vi "Main.vi"(11 "Module Admin":refnum<class "Delacor_lib_QMH_Cloneable Module Admin.lvclass">) -> ()   [LabVIEW 2026, in "Core.lvlib"]
doc: "This template is based off of the Queued Message Handler design pattern and the Queued Message Handler project template that ships with LabVIEW.\n\nThe main difference is that the queue is private to this module and communication between modules is performed via Broadcast and Request events.\n\nRequest events are wrapped in public API methods and are handled in the Event Handling Loop (EHL) of this VI. Any module can register for Broadcast events sent by this module. The EHL generates messages based on user interface actions.\n\nThe Message Handling Loop (MHL) processes messages generated by the EHL, or by other messages. The messages are string values, so new messages can be added easily to the Message Cases case structure in the MHL. Each message cluster can also provide an optional value for Message Data, which is a variant that can be converted to whatever message-specific data is required.\n_____\nBased on DQMH Dev Tools: Project Template 7.1.2.1547."
uses:
  Core.lvlib
  <vilib>/Delacor/Delacor QMH/Libraries/Cloneable Module Admin_class/Delacor_lib_QMH_Cloneable Module Admin.lvclass
  C:/Program Files/National Instruments/LabVIEW 2026/vi.lib/Delacor/Delacor QMH/Libraries/Module Admin_class/Delacor_lib_QMH_Module Admin.lvclass
  Module Data--cluster.ctl
  <vilib>/Delacor/Delacor QMH/Libraries/Message Queue_class/Delacor_lib_QMH_Message Queue.lvclass/Delacor_lib_QMH_Message Queue.ctl
  <vilib>/Delacor/Delacor QMH/Libraries/Cloneable Module Admin_class/Delacor_lib_QMH_Cloneable Module Admin.lvclass/Delacor_lib_QMH_Cloneable Module Admin.ctl
  Stop Argument--cluster.ctl
  <vilib>/Delacor/Delacor QMH/Libraries/Module Admin_class/Delacor_lib_QMH_Module Admin.lvclass/Delacor_lib_QMH_Module Admin.ctl
  LaunchReplayModule Argument--cluster.ctl
  Set Record Run ID Argument--cluster.ctl
  Record Run ID Argument--cluster.ctl
  Record Run ID (Reply Payload)--cluster.ctl
  <vilib>/Utility/miscctls.llb/LVPointTypeDef.ctl
  <vilib>/Delacor/Delacor QMH/Libraries/Message Queue_class/Delacor_lib_QMH_Enqueue Message (Single).vi
  <vilib>/Delacor/Delacor QMH/Libraries/Cloneable Module Admin_class/Delacor_lib_QMH_Get Module ID.vi
  <vilib>/Delacor/Delacor QMH/Libraries/Module Admin_class/Delacor_lib_QMH_Get External Launch.vi
  <vilib>/Delacor/Delacor QMH/Libraries/Message Queue_class/Delacor_lib_QMH_Message Queue.lvclass
  Launcher/Launcher.lvlib
panel:
  out "error out":errorcluster
  out "Status":string
  in  "Simulate EHL Error":bool
  in  "Simulate MHL Error":bool
  # "Other processes communicate with this Module via its Public API (wrappers for its Request Events).\n\nThis Module communicates with other processes via its Broadcast Events.\nAny process that wants to receive these messages can register for this module's Broadcast events."
  # "This template is for the DQMH framework. See the block diagram for more information on how to use this template."
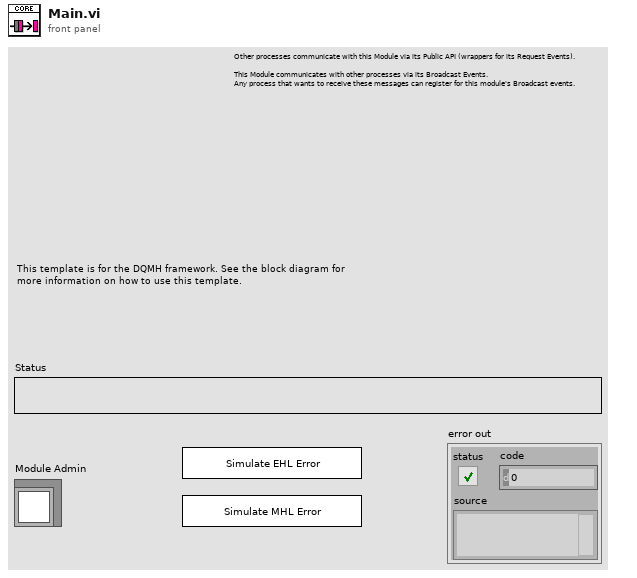
[diagram p1: front panel]
types:
  T1 = typedef "Core.lvlib/Request Events--cluster.ctl" = cluster{"Stop Module":refnum<user-event>, "Show Panel":refnum<user-event>, "Hide Panel":refnum<user-event>, "Show Diagram":refnum<user-event>, "Get Module Execution Status":refnum<user-event>, "Resubscribe to Cloneable":refnum<user-event>, "LaunchReplayModule":refnum<user-event>, "Local Instance":T2, "Record Run ID":refnum<user-event>}
  T2 = typedef "Core.lvlib/Local Instance Request Events--cluster.ctl" = cluster{"Set Record Run ID":refnum<user-event>}
  T3 = typedef "Launcher.lvlib/Broadcast Events--cluster.ctl" = cluster{"Module Did Init":refnum<user-event>, "Status Updated":refnum<user-event>, "Error Reported":refnum<user-event>, "Module Did Stop":refnum<user-event>, "Update Module Execution Status":refnum<user-event>, "Start Capture Detection Loop":refnum<user-event>, "Benchmark Started":refnum<user-event>, "Broadcast number of frames and run ID":refnum<user-event>}
  T4 = typedef "Core.lvlib/Module Data--cluster.ctl" = cluster{"Status":string, "Module ID Recorder":i32, "Record Run ID":string, "Replay Run ID":string}
  T5 = enum32{"invalid lock state", "Not Locked", "Locked (No Password)", "Password-protected"}
  T6 = typedef "Core.lvlib/Stop Argument--cluster.ctl" = cluster{"Module ID":i32, "Origin":string, "Exit via Stop Module Req?":bool, "Wait for Module to stop?":bool}
  T7 = typedef "Core.lvlib/LaunchReplayModule Argument--cluster.ctl" = cluster{"Module ID":i32, "Run ID":string}
  T8 = typedef "Core.lvlib/Set Record Run ID Argument--cluster.ctl" = cluster{"Module ID":i32, "Record Run ID":string}
  T9 = typedef "Core.lvlib/Record Run ID Argument--cluster.ctl" = cluster{"Module ID":i32, "Record Run ID":string, "Wait Notifier":refnum<notifier>, "wait for reply":bool}
  T10 = typedef "LVPointTypeDef.ctl" = cluster{"Horizontal":i16, "Vertical":i16}
  T11 = enum32{"Invalid", "Standard", "Closed", "Hidden", "Minimized", "Maximized"}
  T12 = typedef "Core.lvlib/Record Run ID (Reply Payload)--cluster.ctl" = cluster{"Module ID":i32, "error":errorcluster}
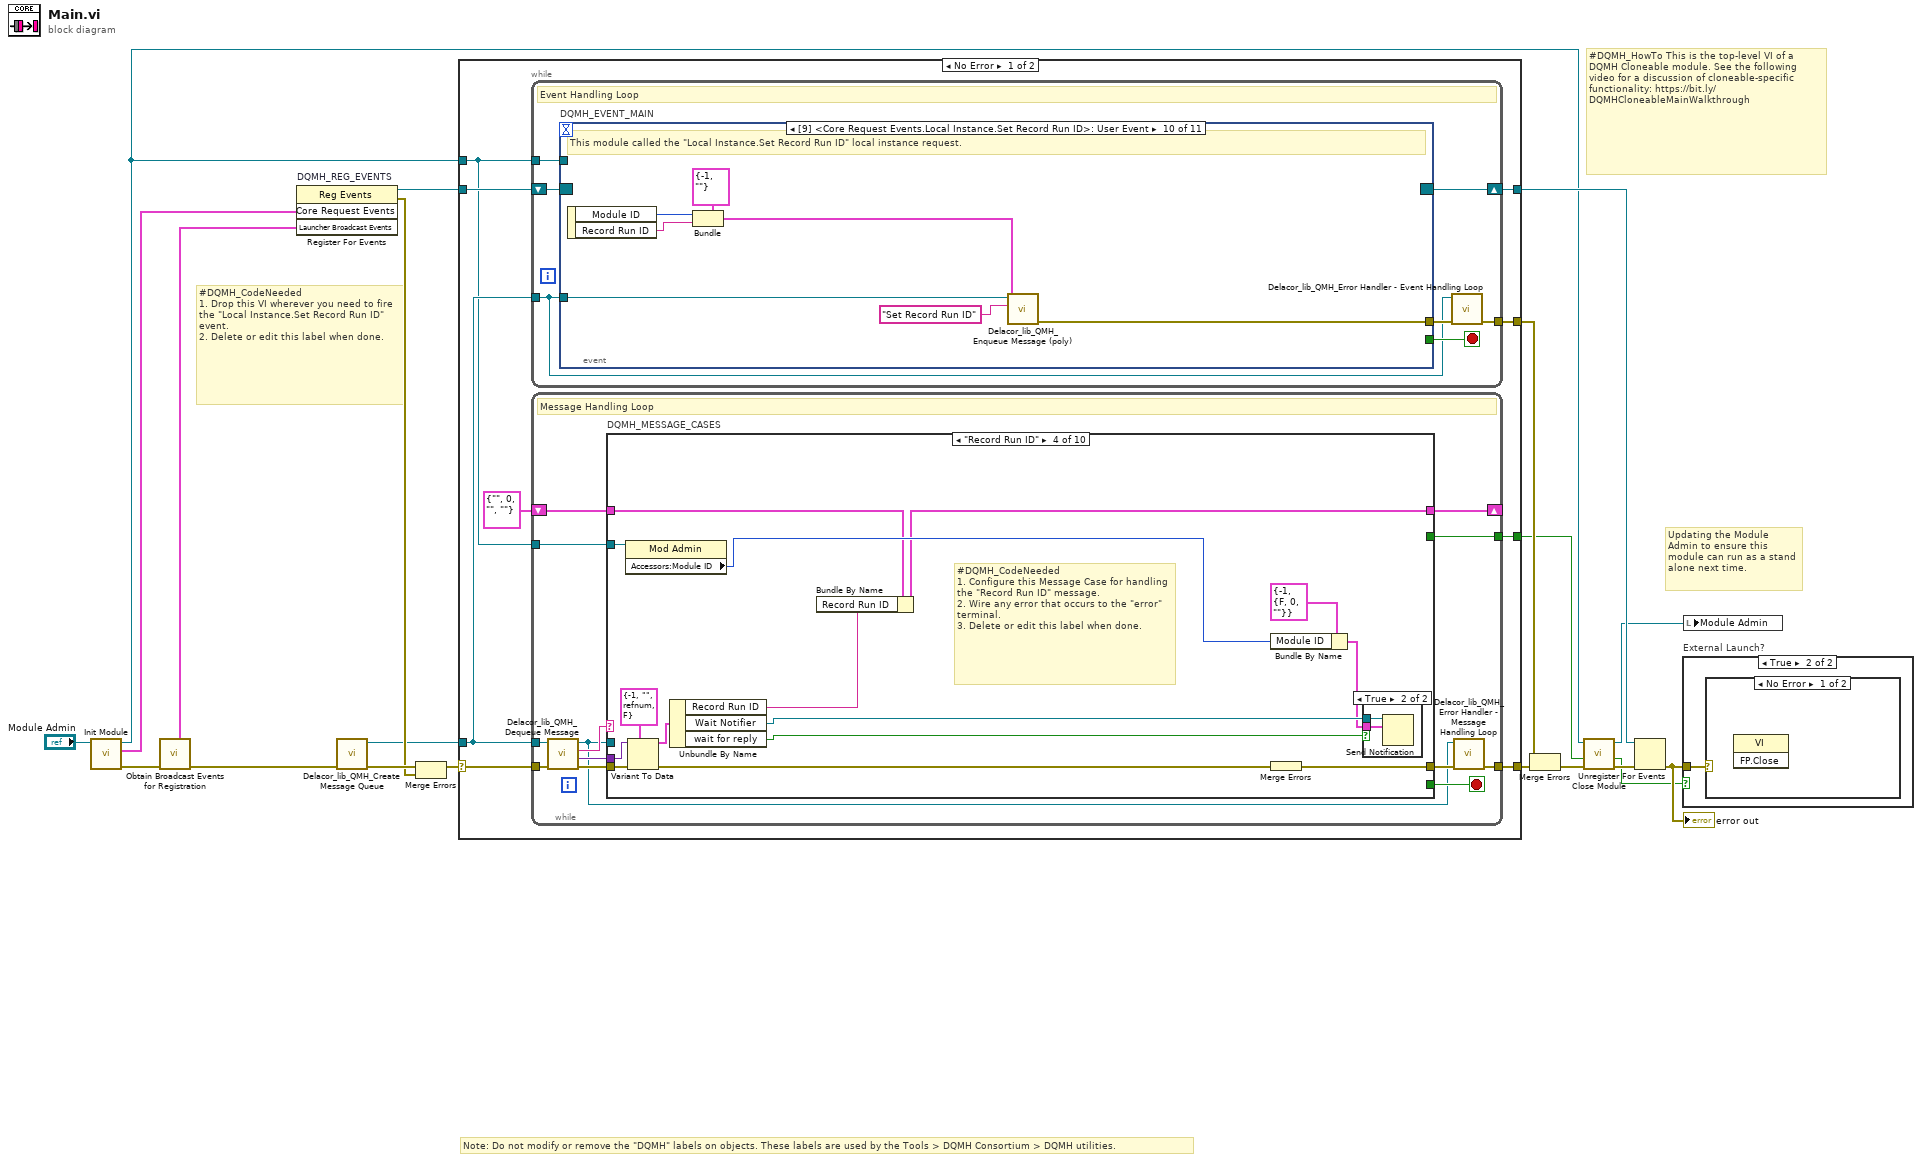
[diagram p0: block diagram]
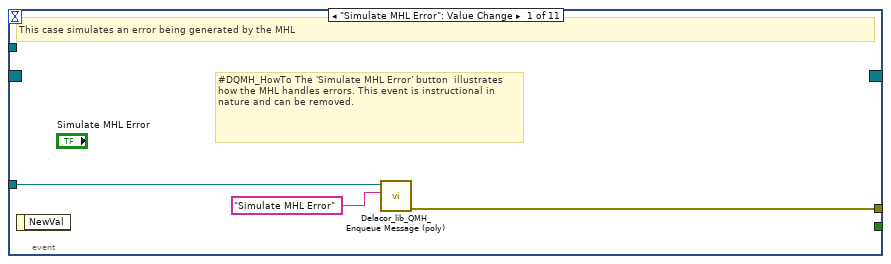
[diagram p2: hidden frame]
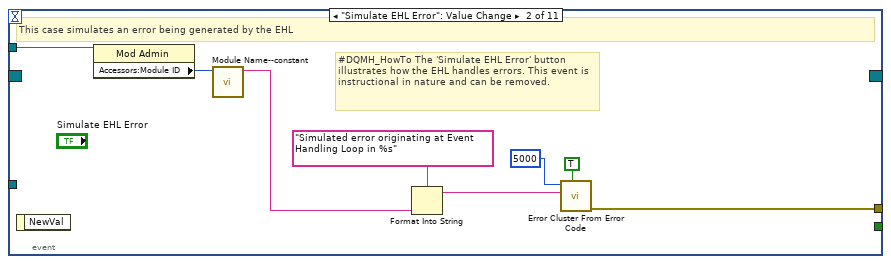
[diagram p3: hidden frame]
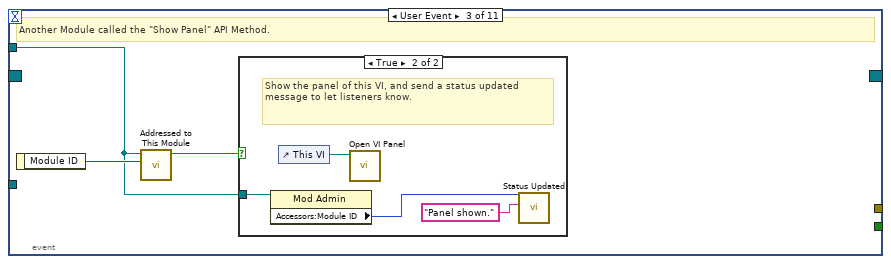
[diagram p4: hidden frame]
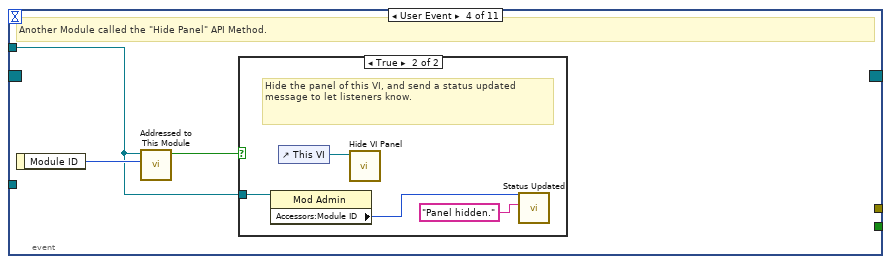
[diagram p6: hidden frame]
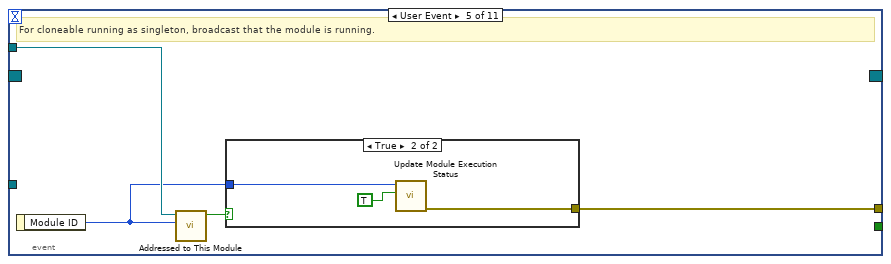
[diagram p8: hidden frame]
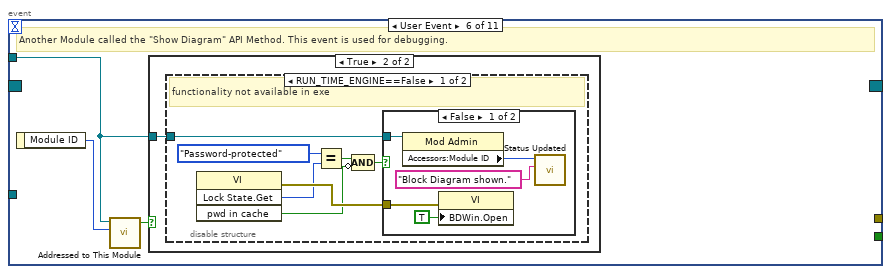
[diagram p10: hidden frame]
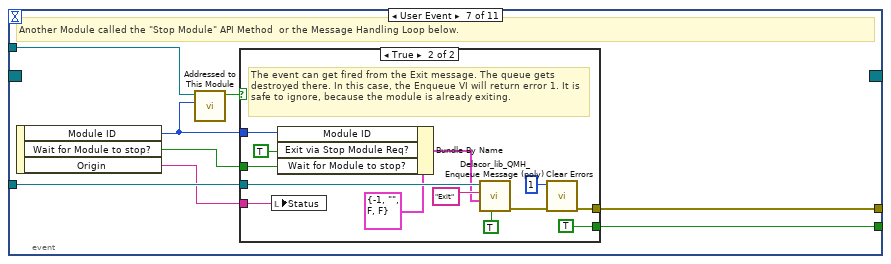
[diagram p14: hidden frame]
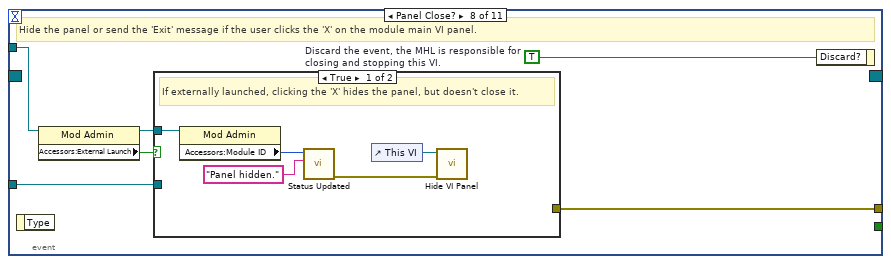
[diagram p16: hidden frame]
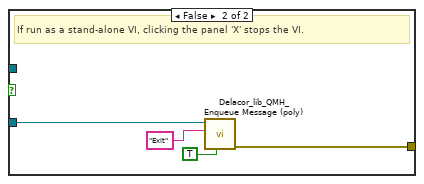
[diagram p17: hidden frame]
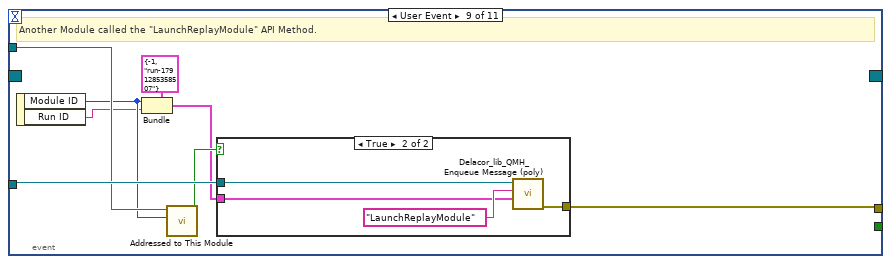
[diagram p18: hidden frame]
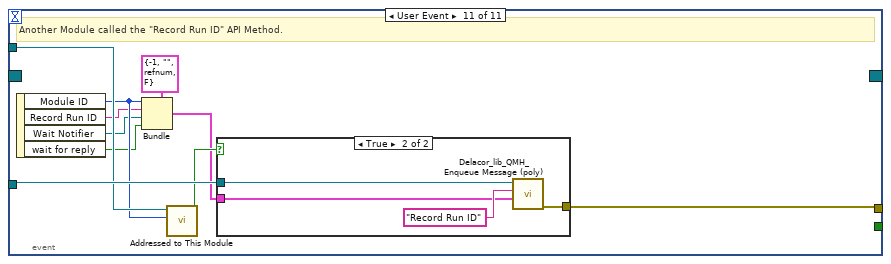
[diagram p20: hidden frame]
diagram:
  # "#DQMH_CodeNeeded\n1. Drop this VI wherever you need to fire the \"Local Instance.Set Record Run ID\" event.\n2. Delete or edit this label when done."
  # "#DQMH_HowTo This is the top-level VI of a DQMH Cloneable module. See the following video for a discussion of cloneable-specific functionality: https://bit.ly/DQMHCloneableMainWalkthrough"
  # "Note: Do not modify or remove the \"DQMH\" labels on objects. These labels are used by the Tools > DQMH Consortium > DQMH utilities."
  # "Updating the Module Admin to ensure this module can run as a stand alone next time."
  n1 = call "Init Module.vi"("Cloneable Module Admin in"="Module Admin") -> ("error out"=w3:errorcluster, "Core Request Events"=w10:T1, "Cloneable Module Admin out"=w7:refnum<class "Delacor_lib_QMH_Cloneable Module Admin.lvclass">)  [unwired: 8 in]
  n2 = call "Obtain Broadcast Events for Registration.vi"("error in"=w3) -> ("error out"=w2:errorcluster, "Launcher Broadcast Events"=w1:T3)  [unwired: 8 in, 1 out]
  n3 = register-events "DQMH_REG_EVENTS"(w10, w1) -> (reference out=w11:refnum<event-registration>, error out=w13:errorcluster)  [unwired: 2 in]
  n4 = call <vilib>:"Delacor_lib_QMH_Create Message Queue.vi"("error in"=w2) -> ("error out"=w15:errorcluster, "Message Queue"=w9:refnum<class "Delacor_lib_QMH_Message Queue.lvclass">)  [unwired: 9 in]
  n5 = Merge Errors(w15, w13) -> (w14:errorcluster)
  n6 = case shown="No Error" w14 {
    selector: w14 -> [w27 w287]
    tunnel: [w29 w286] -> w18
    tunnel: [w26 w285] -> w12
    tunnel: w11 -> [w24 w285]
    tunnel: w9 -> [w23 w278]
    tunnel: [w28 _] -> w19
    tunnel: w7 -> [w22 w281]
    tunnel: [w21 _] -> w5
    frame No Error {
      n7 = while {
        tunnel: w23 -> [w30]
        shift-right: [w33] -> w26
        shift-left: w24 -> [w34]
        tunnel: [w35] -> w28
        tunnel: w22 -> [w31]
        stop <- w32 stop-if-true
        # "Event Handling Loop"
        n8 = event "DQMH_EVENT_MAIN" shown="[9] <Core Request Events.Local Instance.Set Record Run ID>: User Event" {
          selector: w34 -> [_ _ _ _ _ _ _ _ _ _ _]
          dyn-events: [_ _ _ _ _ _ _ _ _ _ _] -> w33
          timeout: _ -> [_ _ _ _ _ _ _ _ _ _ _]
          tunnel: [_ _ _ _ _ _ w88 _ _ _ _] -> w32
          tunnel: w30 -> [w38 _ _ _ _ _ w91 w108 w128 w139 w149]
          tunnel: [w39 w47 _ _ w65 _ w92 w111 w121 w133 w140] -> w36
          tunnel: w31 -> [_ w46 w48 w55 w63 w69 w90 w109 w126 _ w147]
          event "Simulate MHL Error": Value Change {
            # "#DQMH_HowTo The 'Simulate MHL Error' button  illustrates how the MHL handles errors. This event is instructional in nature and can be removed."
            # "This case simulates an error being generated by the MHL"
            n9 = event-data() -> ()  [unwired: 1 in, 1 out]
            n10 = call-poly <vilib>:"Delacor_lib_QMH_Enqueue Message (poly).vi"("Message"="Simulate MHL Error", "Message Queue in"=w38) -> ("error out"=w39:errorcluster)  [unwired: 8 in, 1 out]
          }
          event "Simulate EHL Error": Value Change {
            # "#DQMH_HowTo The 'Simulate EHL Error' button  illustrates how the EHL handles errors. This event is instructional in nature and can be removed."
            # "This case simulates an error being generated by the EHL"
            n11 = event-data() -> ()  [unwired: 1 in, 1 out]
            n12 = property on="Property Node" class="Mod Admin"(reference=w46) -> ("Accessors:Module ID"=w45:i32)  [unwired: 1 in, 2 out]
            n13 = call "Module Name--constant.vi"("Module ID"=w45) -> ("Module Name"=w40:string)  [unwired: 10 in]
            n14 = Format Into String(format string="Simulated error originating at Event Handling Loop in %s", w40) -> (resulting string=w43:string)  [unwired: 2 in, 1 out]
            n15 = call <vilib>:"Error Cluster From Error Code.vi"("show call chain? (False)"=TRUE, "error message (\"\")"=w43, "error code (0)"=5000) -> ("error out"=w47:errorcluster)  [unwired: 6 in]
          }
          event User Event {
            # "Another Module called the \"Show Panel\" API Method."
            n16 = event-data() -> ("Module ID"=w49:i32)  [unwired: 1 in]
            n17 = call "Addressed to This Module.vi"("Module ID from Argument"=w49, "Module Admin"=w48) -> ("Addressed to this instance?"=w50:bool)  [unwired: 8 in, 1 out]
            n18 = case shown="True" w50 {
              tunnel: w48 -> [_ w52]
              frame False {
              }
              frame True {
                # "Show the panel of this VI, and send a status updated message to let listeners know."
                n19 = property on="Property Node" class="Mod Admin"(reference=w52) -> ("Accessors:Module ID"=w51:i32)  [unwired: 1 in, 2 out]
                n20 = control-ref of="This VI"() -> (w54:refnum<vi>)
                n21 = call "Open VI Panel.vi"("VI"=w54) -> ()  [unwired: 10 in, 1 out]
                n22 = call "Status Updated.vi"("Status"="Panel shown." ("format string"), "Module ID"=w51) -> ()  [unwired: 9 in, 1 out]
              }
            }
          }
          event User Event {
            # "Another Module called the \"Hide Panel\" API Method."
            n23 = event-data() -> ("Module ID"=w56:i32)  [unwired: 1 in]
            n24 = call "Addressed to This Module.vi"("Module ID from Argument"=w56, "Module Admin"=w55) -> ("Addressed to this instance?"=w57:bool)  [unwired: 8 in, 1 out]
            n25 = case shown="True" w57 {
              tunnel: w55 -> [_ w59]
              frame False {
              }
              frame True {
                # "Hide the panel of this VI, and send a status updated message to let listeners know."
                n26 = property on="Property Node" class="Mod Admin"(reference=w59) -> ("Accessors:Module ID"=w58:i32)  [unwired: 1 in, 2 out]
                n27 = control-ref of="This VI"() -> (w61:refnum<vi>)
                n28 = call "Hide VI Panel.vi"("VI"=w61) -> ()  [unwired: 10 in, 1 out]
                n29 = call "Status Updated.vi"("Status"="Panel hidden." ("format string"), "Module ID"=w58) -> ()  [unwired: 9 in, 1 out]
              }
            }
          }
          event User Event {
            # "For cloneable running as singleton, broadcast that the module is running."
            n30 = event-data() -> ("Module ID"=w62:i32)  [unwired: 1 in]
            n31 = call "Addressed to This Module.vi"("Module ID from Argument"=w62, "Module Admin"=w63) -> ("Addressed to this instance?"=w64:bool)  [unwired: 8 in, 1 out]
            n32 = case shown="True" w64 {
              tunnel: [_ w68] -> w65
              tunnel: w62 -> [_ w67]
              frame False {
              }
              frame True {
                n33 = call "Update Module Execution Status.vi"("Running?"=TRUE, "Module ID"=w67) -> ("error out"=w68:errorcluster)  [unwired: 9 in]
              }
            }
          }
          event User Event {
            # "Another Module called the \"Show Diagram\" API Method. This event is used for debugging."
            n34 = event-data() -> ("Module ID"=w70:i32)  [unwired: 1 in]
            n35 = call "Addressed to This Module.vi"("Module ID from Argument"=w70, "Module Admin"=w69) -> ("Addressed to this instance?"=w71:bool)  [unwired: 8 in, 1 out]
            n36 = case shown="True" w71 {
              tunnel: w69 -> [_ w72]
              frame False {
              }
              frame True {
                n37 = disable-structure shown="RUN_TIME_ENGINE==False" {
                  disable-tunnel: w72 -> [w73 _]
                  frame condition #0 (active) {
                    # "functionality not available in exe"
                    n38 = invoke on="Invoke Node" class="VI" method="Lock State.Get"() -> (error out=w79:errorcluster, "Get Lock State"=w78:T5, "pwd in cache"=w75:bool)  [unwired: 4 in, 1 out]
                    n39 = Equal?(x=T5."Password-protected", y=w78) -> (x = y?=w76:bool)
                    n40 = Compound Arithmetic op=AND(w76, invert w75) -> (w74:bool)
                    n41 = case shown="False" w74 {
                      tunnel: w79 -> [w84 _]
                      tunnel: w73 -> [w81 _]
                      frame False {
                        n42 = property on="Property Node" class="Mod Admin"(reference=w81) -> ("Accessors:Module ID"=w80:i32)  [unwired: 1 in, 2 out]
                        n43 = property on="Property Node" class="VI"(error in=w84, "BDWin.Open"=TRUE ("Block Diagram Window:Open")) -> ()  [unwired: 1 in, 2 out]
                        n44 = call "Status Updated.vi"("Status"="Block Diagram shown." ("format string"), "Module ID"=w80) -> ()  [unwired: 9 in, 1 out]
                      }
                      frame True {
                        # "Password-protected VI, and the password is not in the cache. Do not show the diagram."
                      }
                    }
                  }
                  frame condition #1 {
                  }
                }
              }
            }
          }
          event User Event {
            # "Another Module called the \"Stop Module\" API Method  or the Message Handling Loop below."
            n45 = event-data() -> ("Module ID"=w86:i32, "Wait for Module to stop?"=w87:bool, "Origin"=w85:string)  [unwired: 1 in]
            n46 = call "Addressed to This Module.vi"("Module ID from Argument"=w86, "Module Admin"=w90) -> ("Addressed to this instance?"=w89:bool)  [unwired: 8 in, 1 out]
            n47 = case shown="True" w89 {
              tunnel: [_ w104] -> w92
              tunnel: w91 -> [_ w100]
              tunnel: [_ TRUE] -> w88
              tunnel: w87 -> [_ w95]
              tunnel: w86 -> [_ w97]
              tunnel: w85 -> [_ w93]
              frame False {
              }
              frame True {
                # "The event can get fired from the Exit message. The queue gets destroyed there. In this case, the Enqueue VI will return error 1. It is safe to ignore, because the module is already exiting."
                n48 = local write "Status"(w93) -> ()
                n49 = Bundle By Name(cluster=T6 {"Module ID"=-1, "Origin"="", "Exit via Stop Module Req?"=FALSE, "Wait for Module to stop?"=FALSE} ("Stop Argument"), "Module ID"=w97, "Exit via Stop Module Req?"=TRUE, "Wait for Module to stop?"=w95) -> (w94:T6)
                n50 = call-poly <vilib>:"Delacor_lib_QMH_Enqueue Message (poly).vi"("Priority Message? (F)"=TRUE, "Message Data"=w94, "Message"="Exit", "Message Queue in"=w100) -> ("error out"=w105:errorcluster)  [unwired: 6 in, 1 out]
                n51 = call <vilib>:"Clear Errors.vi"("error in (no error)"=w105, "specific error code to clear (0: all)"=1) -> ("error out"=w104:errorcluster)  [unwired: 4 in, 1 out]
              }
            }
          }
          event Panel Close? {
            w110 = TRUE  # Discard the event, the MHL is responsible for closing and stopping this VI.
            # "Hide the panel or send the 'Exit' message if the user clicks the 'X' on the module main VI panel."
            n52 = event-data() -> ()  [unwired: 1 in, 1 out]
            n53 = property on="Property Node" class="Mod Admin"(reference=w109) -> (reference out=w106:refnum<class "Delacor_lib_QMH_Cloneable Module Admin.lvclass">, "Accessors:External Launch"=w107:bool)  [unwired: 1 in, 1 out]
            n54 = case shown="True" w107 {
              tunnel: w108 -> [_ w119]
              tunnel: [_ w120] -> w111
              tunnel: w106 -> [w114 _]
              frame True {
                # "If externally launched, clicking the 'X' hides the panel, but doesn't close it."
                n55 = property on="Property Node" class="Mod Admin"(reference=w114) -> ("Accessors:Module ID"=w113:i32)  [unwired: 1 in, 2 out]
                n56 = call "Status Updated.vi"("Status"="Panel hidden." ("format string"), "Module ID"=w113) -> ("error out"=w112:errorcluster)  [unwired: 9 in]
                n57 = control-ref of="This VI"() -> (w116:refnum<vi>)
                n58 = call "Hide VI Panel.vi"("error in"=w112, "VI"=w116) -> ()  [unwired: 9 in, 1 out]
              }
              frame False {
                # "If run as a stand-alone VI, clicking the panel 'X' stops the VI."
                n59 = call-poly <vilib>:"Delacor_lib_QMH_Enqueue Message (poly).vi"("Priority Message? (F)"=TRUE, "Message"="Exit", "Message Queue in"=w119) -> ("error out"=w120:errorcluster)  [unwired: 7 in, 1 out]
              }
            }
            n60 = event-data ("Event Filter Node")("Discard?"=w110) -> ()  [unwired: 1 in, 1 out]
          }
          event User Event {
            # "Another Module called the \"LaunchReplayModule\" API Method."
            n61 = event-data() -> ("Module ID"=w123:i32, "Run ID"=w122:string)  [unwired: 1 in]
            n62 = Bundle(cluster=T7 {"Module ID"=-1, "Run ID"="run-1791285358507"} ("LaunchReplayModule Argument"), "Module ID"=w123, "Run ID"=w122) -> (w124:T7)
            n63 = call "Addressed to This Module.vi"("Module ID from Argument"=w123, "Module Admin"=w126) -> ("Addressed to this instance?"=w127:bool)  [unwired: 8 in, 1 out]
            n64 = case shown="True" w127 {
              tunnel: w128 -> [_ w132]
              tunnel: w124 -> [_ w130]
              tunnel: [_ w129] -> w121
              frame False {
              }
              frame True {
                n65 = call-poly <vilib>:"Delacor_lib_QMH_Enqueue Message (poly).vi"("Message Data"=w130, "Message"="LaunchReplayModule", "Message Queue in"=w132) -> ("error out"=w129:errorcluster)  [unwired: 7 in, 1 out]
              }
            }
          }
          event User Event {
            # "This module called the \"Local Instance.Set Record Run ID\" local instance request."
            n66 = event-data() -> ("Module ID"=w135:i32, "Record Run ID"=w134:string)  [unwired: 1 in]
            n67 = Bundle(cluster=T8 {"Module ID"=-1, "Record Run ID"=""} ("Set Record Run ID Argument"), "Module ID"=w135, "Record Run ID"=w134) -> (w136:T8)
            n68 = call-poly <vilib>:"Delacor_lib_QMH_Enqueue Message (poly).vi"("Message Data"=w136, "Message"="Set Record Run ID", "Message Queue in"=w139) -> ("error out"=w133:errorcluster)  [unwired: 7 in, 1 out]
          }
          event User Event {
            # "Another Module called the \"Record Run ID\" API Method."
            n69 = event-data() -> ("Module ID"=w144:i32, "Record Run ID"=w143:string, "Wait Notifier"=w142:refnum<notifier>, "wait for reply"=w141:bool)  [unwired: 1 in]
            n70 = Bundle(cluster=T9 {"Module ID"=-1, "Record Run ID"="", "Wait Notifier"=refnum, "wait for reply"=FALSE} ("Record Run ID Argument"), "Module ID"=w144, "Record Run ID"=w143, "Wait Notifier"=w142, "wait for reply"=w141) -> (w145:T9)
            n71 = call "Addressed to This Module.vi"("Module ID from Argument"=w144, "Module Admin"=w147) -> ("Addressed to this instance?"=w148:bool)  [unwired: 8 in, 1 out]
            n72 = case shown="True" w148 {
              tunnel: w149 -> [_ w153]
              tunnel: w145 -> [_ w151]
              tunnel: [_ w150] -> w140
              frame False {
              }
              frame True {
                n73 = call-poly <vilib>:"Delacor_lib_QMH_Enqueue Message (poly).vi"("Message Data"=w151, "Message"="Record Run ID", "Message Queue in"=w153) -> ("error out"=w150:errorcluster)  [unwired: 7 in, 1 out]
              }
            }
          }
        }
        n74 = call-dynamic "Delacor_lib_QMH_Error Handler - Event Handling Loop.vi"("error in"=w36, "Message Queue in"=w30) -> ("dup error in"=w35:errorcluster)  [unwired: 8 in, 1 out]
      }
      n75 = while {
        tunnel: w23 -> [w154]
        shift-right: [w161] -> _
        shift-left: T4 {"Status"="", "Module ID Recorder"=0, "Record Run ID"="", "Replay Run ID"=""} ("Data Cluster") -> [w162]
        tunnel: w27 -> [w165]
        tunnel: [w163] -> w29
        tunnel: w22 -> [w156]
        tunnel: [w155] -> w21
        stop <- w160 stop-if-true
        # "Message Handling Loop"
        n76 = call-dynamic "Delacor_lib_QMH_Dequeue Message.vi"("error in"=w165, "Message Queue in"=w154) -> ("error out"=w164:errorcluster, "Message Data"=w158:variant, "Message"=w159:string, "Message Queue out"=w157:refnum<class "Delacor_lib_QMH_Message Queue.lvclass">)  [unwired: 6 in]
        n77 = case "DQMH_MESSAGE_CASES" shown="\"Record Run ID\"" w159 {
          selector: w159 -> [_ _ _ _ _ _ _ _ _ w267]
          tunnel: w157 -> [_ _ _ _ _ _ w222 _ w259 _]
          tunnel: w164 -> [w185 w189 w197 w212 w217 w219 w231 w248 w265 w276]
          tunnel: [w167 w189 w196 w203 w216 w219 w227 w247 w260 w277] -> w166
          tunnel: w162 -> [w177 w188 w192 w200 w215 w218 w226 w245 w249 w274]
          tunnel: [w169 w188 w190 w199 w215 w218 w226 w245 w249 w274] -> w161
          tunnel: [_ _ _ _ _ _ _ _ w258 _] -> w160
          tunnel: w158 -> [_ _ w195 w210 _ _ w225 _ w256 _]
          tunnel: w156 -> [w173 _ _ w201 _ _ w224 w243 w251 w273]
          tunnel: [_ _ _ _ _ _ _ _ w254 _] -> w155
          frame "Initialize" {
            w170 = "Initial Message" ("Initial Message")
            # "#DQMH_CodeNeeded - Initialize the appearance of the front panel."
            # "#DQMH_CodeNeeded - Initialize your state data here."
            # "Initialize - Any operation that needs to be done before the module can receive messages. Synchronize Caller Events.vi will inform Start Module.vi that the module has launched and is ready to receive messages. Module Did Init.vi will broadcast that the module initialized."
            n78 = call "Synchronize Caller Events.vi"("error in"=w185, "Module Admin"=w173) -> ("error out"=w184:errorcluster, "Module Admin out"=w172:refnum<class "Delacor_lib_QMH_Cloneable Module Admin.lvclass">)  [unwired: 8 in]
            n79 = property on="Property Node" class="Mod Admin"(reference=w172) -> ("Accessors:Module ID"=w168:i32, "Accessors:External Launch"=w174:bool)  [unwired: 1 in, 2 out]
            n80 = property on="Pane" class="Pane"("Origin"=T10 {"Horizontal"=0, "Vertical"=0}) -> ()  [unwired: 2 in, 2 out]
            n81 = call "Module Name--constant.vi"("Module ID"=w168) -> ("Module Name"=w181:string)  [unwired: 10 in]
            n82 = property on="Property Node" class="VI"("Front Panel.Title"=w181) -> (reference out=w183:refnum<vi>, error out=w187:errorcluster)  [unwired: 2 in]
            n83 = Select(t=T11."Hidden" ("State"), s=w174, f=T11."Standard" ("State")) -> (s? t:f=w178:T11)
            n84 = call "Module Name--constant.vi"("Module ID"=w168) -> ("Module Name"=w175:string)  [unwired: 10 in]
            n85 = invoke on="Invoke Node" class="VI" method="FP.Open"(reference=w183, error in=w187, "State"=w178) -> (reference out=w182:refnum<vi>, error out=w186:errorcluster)  [unwired: 2 in, 3 out]
            n86 = call "Module Did Init.vi"("error in"=w184, "Initialized?"=TRUE, "Origin"=w175, "Module ID"=w168) -> ("error out"=w167:errorcluster)  [unwired: 7 in]
            n87 = Bundle By Name(cluster=w177, "Status"=w170) -> (w169:T4)
            n88 = invoke on="Invoke Node" class="VI" method="FP.Center"(reference=w182, error in=w186) -> ()  [unwired: 1 in, 3 out]
            "Status" <- w170
          }
          frame "---Module Specific---" {
            # "Separator -- The following cases handle messages specific to this Module."
          }
          frame "Set Record Run ID" {
            # "#DQMH_CodeNeeded\n1. Configure this Message Case for handling the \"Set Record Run ID\" message.\n2. Delete or edit this label when done."
            n89 = Variant To Data(error in=w197, type=T8 {"Module ID"=-1, "Record Run ID"=""} ("Set Record Run ID Argument"), Variant=w195) -> (data=w193:T8, error out=w196:errorcluster)
            n90 = Unbundle By Name(w193) -> ("Record Run ID"=w191:string)
            n91 = Bundle By Name(cluster=w192, "Record Run ID"=w191) -> (w190:T4)
          }
          frame "Record Run ID" {
            # "#DQMH_CodeNeeded\n1. Configure this Message Case for handling the \"Record Run ID\" message.\n2. Wire any error that occurs to the \"error\" terminal.\n3. Delete or edit this label when done."
            n92 = property class="Mod Admin"(reference=w201) -> ("Accessors:Module ID"=w202:i32)  [unwired: 1 in, 2 out]
            n93 = Variant To Data(error in=w212, type=T9 {"Module ID"=-1, "Record Run ID"="", "Wait Notifier"=refnum, "wait for reply"=FALSE} ("Record Run ID Argument"), Variant=w210) -> (data=w208:T9, error out=w211:errorcluster)
            n94 = Unbundle By Name(w208) -> ("Record Run ID"=w198:string, "Wait Notifier"=w207:refnum<notifier>, "wait for reply"=w206:bool)
            n95 = Bundle By Name(cluster=w200, "Record Run ID"=w198) -> (w199:T4)
            n96 = Bundle By Name(cluster=T12 {"Module ID"=-1, "error"={"status"=FALSE, "code"=0, "source"=""}} ("Record Run ID (Reply Payload)"), "Module ID"=w202) -> (w205:T12)
            n97 = Merge Errors(w211) -> (w203:errorcluster)
            n98 = case "DQMH_FIRE_NOTIFIER" shown="True" w206 {
              tunnel: w207 -> [_ w214]
              tunnel: w205 -> [_ w213]
              frame False {
              }
              frame True {
                n99 = Send Notification(notification=w213, notifier=w214) -> ()  [unwired: 1 in, 2 out]
              }
            }
          }
          frame "---Copy This Frame---" {
            # "Duplicate this frame when creating new messages.  Change this comment in the duplicated frame to describe this message."
            n100 = Merge Errors(w217) -> (w216:errorcluster)
          }
          frame "---Exit and Error Handling---" {
            # "Separator - the following cases handle errors and exit messages."
          }
          frame "Error" {
            # "#DQMH_CodeRecommended - If the module is running in standalone mode (External Launch = FALSE), this code will pop up an error dialog and call the 'Exit' message if an error occurs. Add more fine-grained error management here."
            # "Error - Check the error message data and respond accordingly. This message is sent by the \"Error Handler\" VIs at the end of each loop in this application."
            n101 = property on="Property Node" class="Mod Admin"(reference=w224) -> ("Accessors:External Launch"=w223:bool, "Accessors:Module ID"=w221:i32)  [unwired: 1 in, 2 out]
            n102 = Variant To Data(error in=w231, type=errorcluster {"status"=FALSE, "code"=0, "source"=""} ("error constant"), Variant=w225) -> (data=w220:errorcluster, error out=w229:errorcluster)
            n103 = local write "error out"(w220) -> ()
            n104 = call "Error Reported.vi"("Error"=w220, "Module ID"=w221) -> ()  [unwired: 9 in, 1 out]
            n105 = case shown="False" w223 {
              tunnel: [w236 _] -> w228
              tunnel: w222 -> [w234 _]
              tunnel: w220 -> [w235 _]
              frame False {
                n106 = disable-structure shown="Default" {
                  disable-tunnel: w235 -> [w237 _]
                  frame condition #0 (active) {
                    # "If the module is running standalone, then pop up an error dialog and call the \"Exit\" message."
                    n107 = call <vilib>:"Simple Error Handler.vi"("error in (no error)"=w237) -> ()  [unwired: 4 in, 5 out]
                  }
                  frame condition #1 {
                    # "To prevent the Simple Error Handler VI from being loaded (e.g. when deploying to a Real-Time target), add the Conditional Disable Symbol \"DQMH_Disable_SEH\" to your project and set it to TRUE."
                  }
                }
                n108 = call-poly <vilib>:"Delacor_lib_QMH_Enqueue Message (poly).vi"("Priority Message? (F)"=TRUE, "Message"="Exit", "Message Queue in"=w234) -> ("error out"=w236:errorcluster)  [unwired: 7 in, 1 out]
              }
              frame True {
                # "If the module was launched externally, calling the Error Reported broadcast VI is the only action performed by the \"Error\" message. The module's caller can then process the error appropriately."
              }
            }
            n109 = Merge Errors(w229, w228) -> (w227:errorcluster)
          }
          frame "Simulate MHL Error" {
            # "#DQMH_HowTo The 'Simulate MHL Error' button  illustrates how the MHL handles errors. This event is instructional in nature and can be removed."
            # "Simulate an error occurring at the MHL"
            n110 = property on="Property Node" class="Mod Admin"(reference=w243) -> ("Accessors:Module ID"=w244:i32)  [unwired: 1 in, 2 out]
            n111 = call "Module Name--constant.vi"("Module ID"=w244) -> ("Module Name"=w239:string)  [unwired: 10 in]
            n112 = Format Into String(format string="Simulated error originating at Message Handling Loop in %s", w239) -> (resulting string=w240:string)  [unwired: 2 in, 1 out]
            n113 = call <vilib>:"Error Cluster From Error Code.vi"("show call chain? (False)"=TRUE, "error message (\"\")"=w240, "error code (0)"=5001) -> ("error out"=w246:errorcluster)  [unwired: 6 in]
            n114 = Merge Errors(w248, w246) -> (w247:errorcluster)
          }
          frame "Exit" {
            (unwired) TRUE ("Wait for Module to stop? (F)")
            w257 = 91  # 91: not all Exit messages will have an argument
            w258 = TRUE  # Stop the VI
            # "Release the message queue reference"
            # "#DQMH_CodeNeeded - Add any required cleanup code here."
            # "Exit - Exit the application."
            n115 = Unbundle By Name(w249) -> ()  [unwired: 1 out]
            n116 = Variant To Data(error in=w265, type=T6 {"Module ID"=-1, "Origin"="", "Exit via Stop Module Req?"=FALSE, "Wait for Module to stop?"=FALSE} ("Stop Argument"), Variant=w256) -> (data=w253:T6, error out=w261:errorcluster)
            n117 = call <vilib>:"Clear Errors.vi"("error in (no error)"=w261, "specific error code to clear (0: all)"=w257) -> ("error out"=w264:errorcluster)  [unwired: 4 in, 1 out]
            n118 = property on="Property Node" class="Mod Admin"(reference=w251) -> ("Accessors:Module ID"=w250:i32)  [unwired: 1 in, 2 out]
            n119 = call-dynamic "Delacor_lib_QMH_Release Message Queue.vi"("error in"=w264, "Message Queue"=w259) -> ("error out"=w263:errorcluster)  [unwired: 9 in]
            n120 = control-ref of="This VI"() -> (w252:refnum<vi>)
            n121 = call "Handle Exit.vi"("Stop Argument"=w253, "Module Admin in"=w251, "VI reference"=w252) -> ("error out"=w262:errorcluster, "Wait for Stop?"=w254:bool)  [unwired: 7 in]
            n122 = Merge Errors(w263, w262) -> (w260:errorcluster)
            n123 = call "Error Reported.vi"("Error"=w260, "Module ID"=w250) -> ()  [unwired: 9 in, 1 out]
          }
          frame Default {
            # "'Default' case only runs if there is a message that isn't defined in any of the other cases.  Output a programming error."
            n124 = property on="Property Node" class="Mod Admin"(reference=w273) -> ("Accessors:Module ID"=w272:i32)  [unwired: 1 in, 2 out]
            n125 = call "Module Name--constant.vi"("Module ID"=w272) -> ("Module Name"=w266:string)  [unwired: 10 in]
            n126 = Format Into String(format string="The invalid message string \"%s\" was received in the Message Handling Loop for module \"%s\".", w267, w266) -> (resulting string=w269:string)  [unwired: 2 in, 1 out]
            n127 = call <vilib>:"Error Cluster From Error Code.vi"("show call chain? (False)"=TRUE, "error message (\"\")"=w269, "error code (0)"=1) -> ("error out"=w275:errorcluster)  [unwired: 6 in]
            n128 = Merge Errors(w276, w275) -> (w277:errorcluster)
          }
        }
        n129 = call-dynamic "Delacor_lib_QMH_Error Handler - Message Handling Loop.vi"("error in"=w166, "Message Queue in"=w157) -> ("dup error in"=w163:errorcluster)  [unwired: 8 in, 1 out]
      }
    }
    frame Error {
      n130 = call "Synchronize Caller Events.vi"("Module Admin"=w281) -> ("Module Admin out"=w280:refnum<class "Delacor_lib_QMH_Cloneable Module Admin.lvclass">)  [unwired: 9 in, 1 out]
      n131 = property on="Property Node" class="Mod Admin"(reference=w280) -> ("Accessors:Module ID"=w279:i32)  [unwired: 1 in, 2 out]
      n132 = call-dynamic "Delacor_lib_QMH_Release Message Queue.vi"("error in"=w287, "Message Queue"=w278) -> ("error out"=w286:errorcluster)  [unwired: 9 in]
      n133 = call "Module Name--constant.vi"("Module ID"=w279) -> ("Module Name"=w284:string)  [unwired: 10 in]
      n134 = Format Into String(format string="An error occurred during initialization. %s is no longer running.", w284) -> (resulting string=w282:string)  [unwired: 2 in, 1 out]
      n135 = call "Error Reported.vi"("Additional Information"=w282, "Error"=w286, "Module ID"=w279) -> ()  [unwired: 8 in, 1 out]
    }
  }
  n136 = Merge Errors(w19, w18) -> (w20:errorcluster)
  n137 = call "Close Module.vi"("error in"=w20, "Wait for stop?"=w5, "Module Admin in"=w7) -> ("error out"=w17:errorcluster, "External Launch"=w4:bool, "Module Admin out"=w6:refnum<class "Delacor_lib_QMH_Cloneable Module Admin.lvclass">)  [unwired: 6 in]
  n138 = Unregister For Events(event registration refnum=w12, error in=w17) -> (error out=w16:errorcluster)
  "error out" <- w16
  n139 = case "External Launch?" shown="True" w4 {
    tunnel: w16 -> [_ w288]
    frame False {
    }
    frame True {
      n140 = case shown="No Error" w288 {
        frame No Error {
          n141 = invoke class="VI" method="FP.Close"() -> ()  [unwired: 3 in, 3 out]
        }
        frame Error {
          n142 = disable-structure shown="Default" {
            frame condition #0 (active) {
              n143 = invoke class="VI" method="FP.Open"("Activate"=TRUE ("Activate?")) -> ()  [unwired: 4 in, 5 out]
            }
            frame condition #1 {
              # "Don't show panel on error if running inside a built EXE."
            }
          }
        }
      }
    }
  }
  n144 = local write "Module Admin"(w6) -> ()
